vi "Own20261012_GetInvokeInfo.vi"() -> ()   [LabVIEW 2024]
uses:
  <vilib>/_script/All Supported PropertiesOrMethods TypeDefs/ASPM_UniqueIDStringDatanameShortnameLongname.ctl
  <vilib>/_script/All Supported PropertiesOrMethods TypeDefs/ASPM_ArrayOfUniqueIDStringDatanameShortnameLongname.ctl
panel:
  out "supported_methods":T1 caption="全部支持方法"
  out "method":T2 caption="方法"
  out "error out":errorcluster caption="错误输出"
  out "class_name":string
  in  "invoke_id":u32
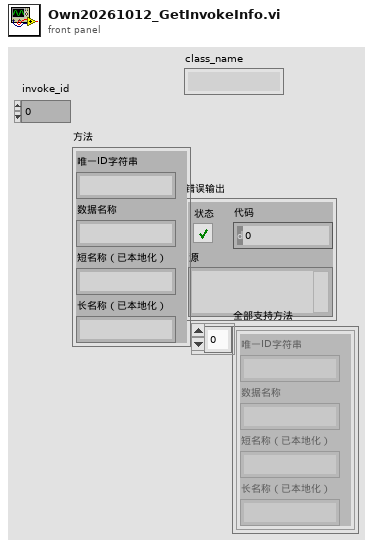
[diagram p1: front panel]
types:
  T1 = typedef "ASPM_ArrayOfUniqueIDStringDatanameShortnameLongname.ctl" = T2[]
  T2 = typedef "ASPM_UniqueIDStringDatanameShortnameLongname.ctl" = cluster{"Unique ID string":string, "Data name":string, "Short name (localized)":string, "Long name (localized)":string}
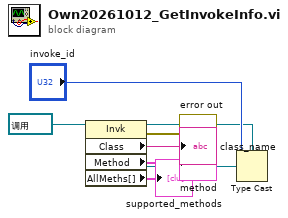
[diagram p0: block diagram]
diagram:
  n1 = Type Cast(type=refnum<vi> refnum ("引用"), x="invoke_id") -> (*(type *) &x=w5:refnum<vi>)
  n2 = property class="Invk"(reference=w5) -> (error out=→"error out":errorcluster, "Class"=→"class_name":string, "Method"=→"method":T2, "AllMeths[]"=→"supported_methods":T1)  [unwired: 1 in, 1 out]
